vi "IVCentral Heater Global.vi"() -> ()   [LabVIEW 2026]
panel:
  in  "I V  Central heater":dbl[](array[numeric])
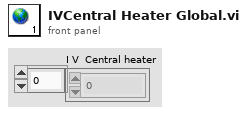
[diagram p1: front panel]
diagram:
